vi "Find OOB Server Ports.vi"(8 "error in":errorcluster) -> (3 "Ports":u16[](array[numeric]))   [LabVIEW 2026]
uses:
  <vilib>/Utility/error.llb/Trim Whitespace One-Sided.vi
panel:
  out "element":string
  out "string array":string[](array[string])
  out "standard output":string
  out "netstat":T1(array[cluster])
  out "standard error":string
  out "return code":i32
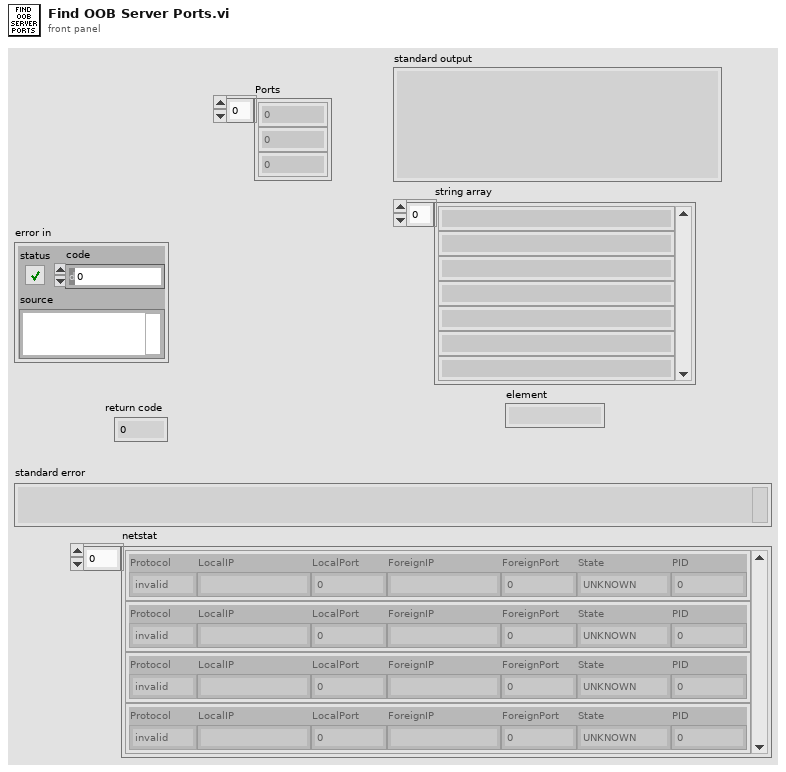
[diagram p1: front panel]
types:
  T1 = cluster{"Protocol":enum16{"invalid", "tcp", "udp", "icmp", "ip", "tcpv6", "udpv6", "icmpv6", "ipv6"}, "LocalIP":string, "LocalPort":u16, "ForeignIP":string, "ForeignPort":u16, "State":enum8{"UNKNOWN", "LISTEN", "ESTABLISHED", "SYN_SENT", "SYN_RECV", "LAST_ACK", "CLOSE_WAIT", "TIME_WAIT", "CLOSED", "CLOSING", "FIN_WAIT1", "FIN_WAIT2"}, "PID":u16}[]
  T2 = enum8{"UNKNOWN", "LISTEN", "ESTABLISHED", "SYN_SENT", "SYN_RECV", "LAST_ACK", "CLOSE_WAIT", "TIME_WAIT", "CLOSED", "CLOSING", "FIN_WAIT1", "FIN_WAIT2"}
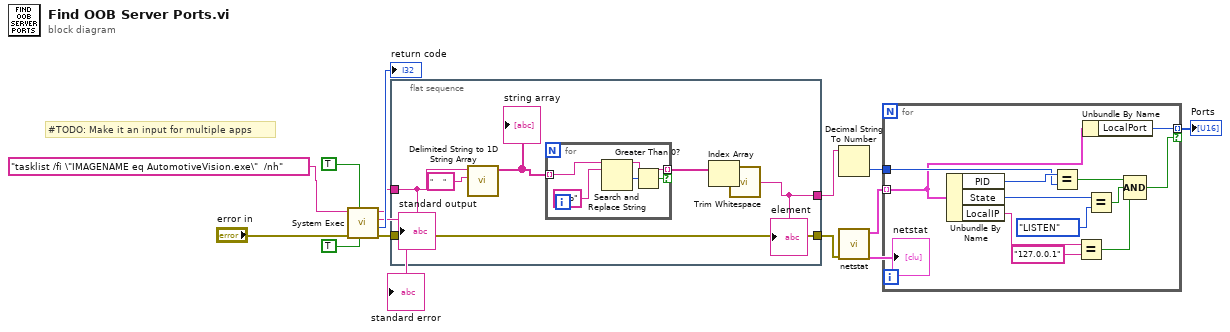
[diagram p0: block diagram]
diagram:
  # "#TODO: Make it an input for multiple apps"
  n1 = call <vilib>:"System Exec.vi"("run minimized? (F)"=TRUE, "wait until completion? (T)"=TRUE, "error in (no error)"="error in", "command line"="tasklist /fi \"IMAGENAME eq AutomotiveVision.exe\"  /nh") -> ("error out"=w9:errorcluster, "return code"=→"return code":i32, "standard error"=→"standard error":string, "standard output"=w7:string)  [unwired: 4 in]
  n2 = flat-sequence {
    tunnel: w7 -> [w20]
    tunnel: [w14] -> w8
    tunnel: w9 -> [w17]
    tunnel: [w17] -> w4
    frame #0 {
      n3 = call <vilib>:"Delimited String to 1D String Array.vi"("delimiter"="     ", "delimited string"=w20) -> ("string array"=w16:string[])  [unwired: 9 in]
      "string array" <- w16
      n4 = for {
        tunnel: w16 -> [w24] mode=indexing
        tunnel: [w23] -> w15 mode=indexing if=w21
        n5 = Search and Replace String(input string=w24, search string="Tcp") -> (result string=w23:string, offset past replacement=w22:i32)  [unwired: 6 in, 2 out]
        n6 = Greater Than 0?(x=w22) -> (x > 0?=w21:bool)
      }
      n7 = Index Array(array=w15) -> (element=w18:string)  [unwired: 1 in]
      n8 = call <vilib>:"Trim Whitespace.vi"("string"=w18) -> ("trimmed string"=w14:string)  [unwired: 1 in]
      "element" <- w14
      "standard output" <- w20
    }
  }
  n9 = Decimal String To Number(string=w8) -> (number=w6:i32)  [unwired: 2 in, 1 out]
  n10 = call "netstat.vi"("error in (no error)"=w4) -> ("netstat"=w5:T1)  [unwired: 9 in, 1 out]
  "netstat" <- w5
  n11 = for {
    tunnel: w5 -> [w28] mode=indexing
    tunnel: w6 -> [w36]
    tunnel: [w27] -> w3 mode=indexing if=w26
    n12 = Unbundle By Name(w28) -> ("PID"=w37:u16, "State"=w34:T2, "LocalIP"=w31:string)
    n13 = Equal?(x=w37, y=w36) -> (x = y?=w35:bool)
    n14 = Equal?(x=w31, y="127.0.0.1") -> (x = y?=w29:bool)
    n15 = Unbundle By Name(w28) -> ("LocalPort"=w27:u16)
    n16 = Equal?(x=w34, y=T2."LISTEN") -> (x = y?=w32:bool)
    n17 = Compound Arithmetic op=AND(w35, w32, w29) -> (w26:bool)
  }
  "Ports" <- w3
